vi "KalmanFilter_SetXHat.vi"(9 "xHat":T1, 11 "in KalmanFilter":T2) -> (0 "Size Coerced":bool, 3 "out KalmanFilter":T2)   [LabVIEW 2019, in "Trajectory_Library.lvlib"]
doc: "Set initial state estimate x-hat.\n \nInputs:\n - inKalmanFilter -- filter data cluster\n - xhat -- The state estimate x-hat.\n \nOutputs:\n - outKalmanFilter -- updated filter data cluster\n - sizeCoerced -- If TRUE, an unexpected error occured with the size of the input xHat"
uses:
  Trajectory_Library.lvlib
  <vilib>/Analysis/Matrix/Datatypes/RealMatrix.ctl
  <vilib>/Analysis/Matrix/NI_Matrix.lvlib
  TypeDef/LINEAR_SYSTEM.ctl
  TypeDef/KALMAN_FILTER.ctl
panel:
  # "Steady State Gain  \n<States,Outputs>"
  # "State Estimate <Statess,1>"
  # "<States,States>"
  # "<States,Inputs>"
  # "<Outputs,States>"
  # "<Outputs,Inputs>"
  # "Steady State Gain  \n<States,Outputs>"
  # "State Estimate <Statess,1>"
  # "<States,States>"
  # "<States,Inputs>"
  # "<Outputs,States>"
  # "<Outputs,Inputs>"
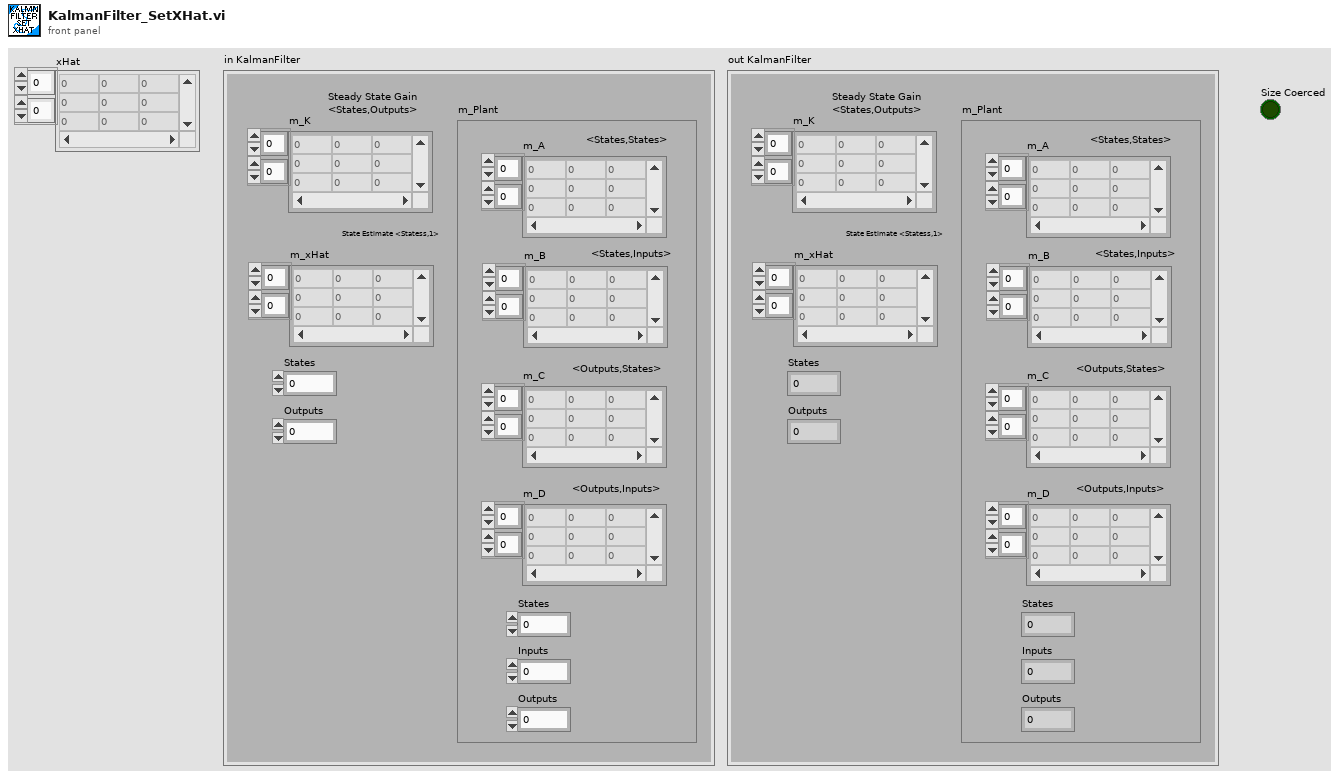
[diagram p1: front panel]
types:
  T1 = typedef "NI_Matrix.lvlib/RealMatrix.ctl" = dbl[][]
  T2 = typedef "Trajectory_Library.lvlib/KALMAN_FILTER.ctl" = cluster{"m_K":T1, "m_xHat":T1, "States":i32, "Outputs":i32, "m_Plant":T3}
  T3 = typedef "Trajectory_Library.lvlib/LINEAR_SYSTEM.ctl" = cluster{"m_A":T1, "m_B":T1, "m_C":T1, "m_D":T1, "States":i32, "Inputs":i32, "Outputs":i32}
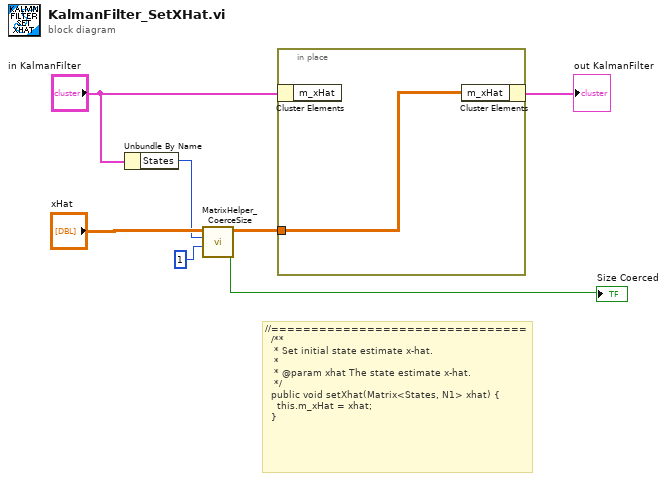
[diagram p0: block diagram]
diagram:
  # "//================================\n  /**\n   * Set initial state estimate x-hat.\n   *\n   * @param xhat The state estimate x-hat.\n   */\n  public void setXhat(Matrix<States, N1> xhat) {\n    this.m_xHat = xhat;\n  }"
  n1 = Unbundle By Name("in KalmanFilter") -> ("States"=w3:i32)
  n2 = call "MatrixHelper_CoerceSize.vi"("Columns"=1, "Rows"=w3, "input matrix"="xHat") -> ("Coerced"=→"Size Coerced":bool, "output matrix"=w4:T1)  [unwired: 7 in]
  n3 = in-place {
    in-place-border: w4 -> [w8]
    n4 = in-place-cluster #1("in KalmanFilter") -> ()  [unwired: 1 out]
    n5 = in-place-cluster #1("m_xHat"=w8) -> (→"out KalmanFilter":T2)
  }
